vi "CSE ISP - options.vi"(8 "cmd":enum16{"get", "default"}(ring), 9 "enable menu (T)":bool=TRUE, 10 "item subtag":string, 11 "ISP menu":refnum<k9>) -> (0 "error out":errorcluster, 1 "VM params":T2, 2 "load FuncVIs":u32(ring)=2 items=["don't load", "load", "load & test"], 3 "dup ISP menu":refnum<k9>, 4 "Parse params":T4={"AutoParse"=TRUE, "GroupStm"=FALSE, "ErrSrcMaxLen"=180}, 5 "test syntax only":bool, 6 "misc params":T1, 7 "Exec params":T3={"pause counter"=1000, "pause, ms"=0, "autoVar"=TRUE, "enCpx"=TRUE})   [LabVIEW 2021]
doc: "::: CalcExpress Toolkit :::\nCopyright (c) 2000-2026 Konstantin Shifershteyn. All rights reserved."
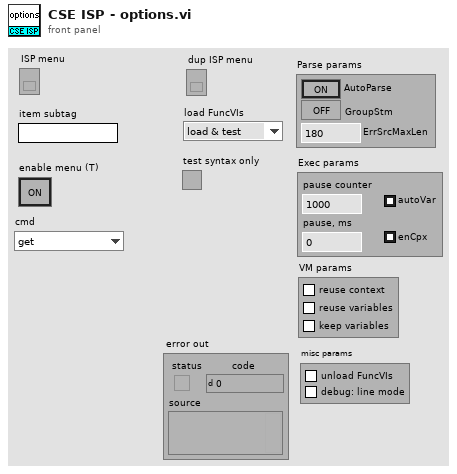
[diagram p1: front panel]
types:
  T1 = cluster{"unload FuncVIs":bool, "debug: line mode":bool}
  T2 = cluster{"reuse context":bool, "reuse variables":bool, "keep variables":bool}
  T3 = cluster{"pause counter":i32, "pause, ms":i32, "autoVar":bool, "enCpx":bool}
  T4 = cluster{"AutoParse":bool, "GroupStm":bool, "ErrSrcMaxLen":i32}
  T5 = cluster{i32, i32, "checked":bool, "checked":bool}
  T6 = cluster{"checked":bool, "checked":bool, "checked":bool}
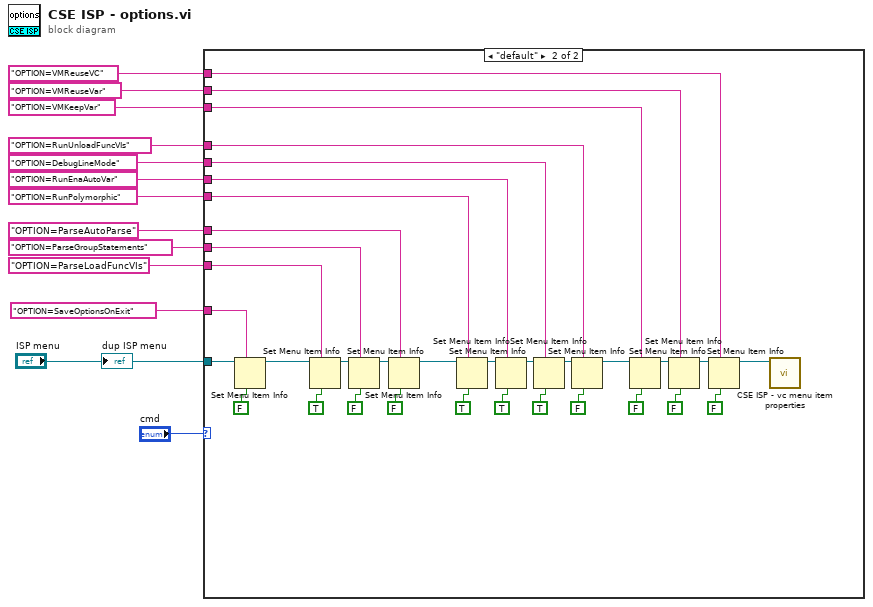
[diagram p0: block diagram]
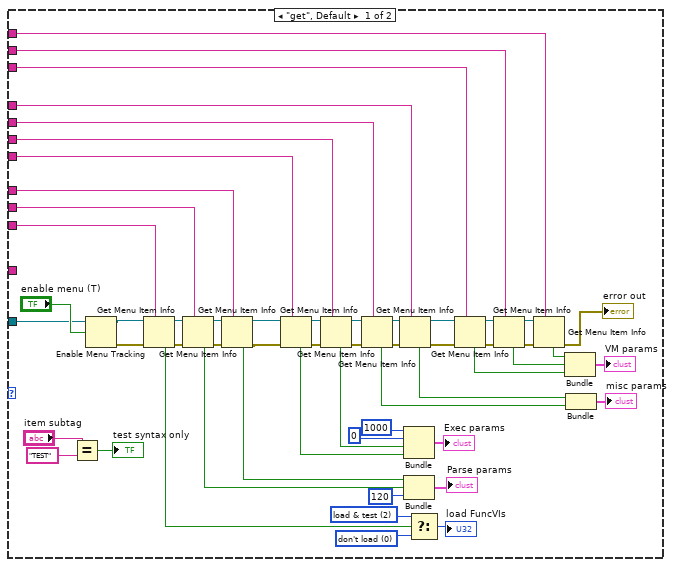
[diagram p2: hidden frame]
diagram:
  n1 = case shown="\"default\"" "cmd" {
    tunnel: "OPTION=RunUnloadFuncVIs" ("item tag") -> [w69 w103]
    tunnel: "OPTION=ParseGroupStatements" ("item tag") -> [w67 w101]
    tunnel: "OPTION=ParseAutoParse" ("item tag") -> [w66 w100]
    tunnel: "OPTION=RunPolymorphic" ("item tag") -> [w56 w99]
    tunnel: "OPTION=RunEnaAutoVar" ("item tag") -> [w55 w98]
    tunnel: "OPTION=ParseLoadFuncVIs" ("item tag") -> [w50 w102]
    tunnel: "ISP menu" -> [w43 w77]
    tunnel: "OPTION=SaveOptionsOnExit" ("item tag") -> [_ w87]
    tunnel: "OPTION=VMReuseVC" ("item tag") -> [w35 w81]
    tunnel: "OPTION=VMReuseVar" ("item tag") -> [w34 w82]
    tunnel: "OPTION=VMKeepVar" ("item tag") -> [w33 w83]
    tunnel: "OPTION=DebugLineMode" ("item tag") -> [w23 w73]
    frame "get", Default {
      w44 = u32 2 items=["don't load", "load", "load & test"] ("load FuncVIs")
      w45 = u32 0 items=["don't load", "load", "load & test"] ("load FuncVIs")
      n2 = Equal?(x="item subtag", y="TEST") -> (x = y?=→"test syntax only":bool)
      n3 = Enable Menu Tracking(3:"enable menu (T)", 4:w43) -> (0:w29:errorcluster, 1:w30:refnum<k9>)  [unwired: 1 in]
      n4 = Get Menu Item Info(7:w50, 8:w29, 11:w30) -> (0:w48:errorcluster, 3:w49:refnum<k9>, 4:w47:bool)  [unwired: 4 out]
      n5 = Get Menu Item Info(7:w67, 8:w48, 11:w49) -> (0:w58:errorcluster, 3:w68:refnum<k9>, 4:w63:bool)  [unwired: 4 out]
      n6 = Get Menu Item Info(7:w66, 8:w58, 11:w68) -> (0:w14:errorcluster, 3:w15:refnum<k9>, 4:w64:bool)  [unwired: 4 out]
      n7 = Get Menu Item Info(7:w56, 8:w14, 11:w15) -> (0:w57:errorcluster, 3:w59:refnum<k9>, 4:w52:bool)  [unwired: 4 out]
      n8 = Get Menu Item Info(7:w55, 8:w57, 11:w59) -> (0:w25:errorcluster, 3:w24:refnum<k9>, 4:w53:bool)  [unwired: 4 out]
      n9 = Get Menu Item Info(7:w23, 8:w25, 11:w24) -> (0:w18:errorcluster, 3:w19:refnum<k9>, 4:w21:bool)  [unwired: 4 out]
      n10 = Get Menu Item Info(7:w69, 8:w18, 11:w19) -> (0:w17:errorcluster, 3:w16:refnum<k9>, 4:w22:bool)  [unwired: 4 out]
      n11 = Bundle(1000, 0, "checked"=w53, "checked"=w52) -> (→"Exec params":T5)  [unwired: 1 in]
      n12 = Bundle("checked"=w64, "checked"=w63, 120) -> (→"Parse params":cluster{"checked":bool, "checked":bool, i32})  [unwired: 1 in]
      n13 = Select(t=w44, s=w47, f=w45) -> (s? t:f=→"load FuncVIs":u32)
      n14 = Get Menu Item Info(7:w33, 8:w17, 11:w16) -> (0:w40:errorcluster, 3:w42:refnum<k9>, 4:w36:bool)  [unwired: 4 out]
      n15 = Get Menu Item Info(7:w34, 8:w40, 11:w42) -> (0:w39:errorcluster, 3:w41:refnum<k9>, 4:w37:bool)  [unwired: 4 out]
      n16 = Get Menu Item Info(7:w35, 8:w39, 11:w41) -> (0:→"error out":errorcluster, 4:w38:bool)  [unwired: 5 out]
      n17 = Bundle("checked"=w38, "checked"=w37, "checked"=w36) -> (→"VM params":T6)  [unwired: 1 in]
      n18 = Bundle("checked"=w22, "checked"=w21) -> (→"misc params":cluster{"checked":bool, "checked":bool})  [unwired: 1 in]
    }
    frame "default" {
      n19 = Set Menu Item Info(6:FALSE ("checked"), 7:w87, 11:w77) -> (3:w76:refnum<k9>)  [unwired: 4 in, 1 out]
      n20 = Set Menu Item Info(6:TRUE ("checked"), 7:w102, 11:w76) -> (3:w97:refnum<k9>)  [unwired: 4 in, 1 out]
      n21 = Set Menu Item Info(6:FALSE ("checked"), 7:w101, 11:w97) -> (3:w96:refnum<k9>)  [unwired: 4 in, 1 out]
      n22 = Set Menu Item Info(6:FALSE ("checked"), 7:w100, 11:w96) -> (3:w71:refnum<k9>)  [unwired: 4 in, 1 out]
      n23 = Set Menu Item Info(6:TRUE ("checked"), 7:w99, 11:w71) -> (3:w95:refnum<k9>)  [unwired: 4 in, 1 out]
      n24 = Set Menu Item Info(6:TRUE ("checked"), 7:w98, 11:w95) -> (3:w74:refnum<k9>)  [unwired: 4 in, 1 out]
      n25 = Set Menu Item Info(6:TRUE ("checked"), 7:w73, 11:w74) -> (3:w72:refnum<k9>)  [unwired: 4 in, 1 out]
      n26 = Set Menu Item Info(6:FALSE ("checked"), 7:w103, 11:w72) -> (3:w70:refnum<k9>)  [unwired: 4 in, 1 out]
      n27 = Set Menu Item Info(6:FALSE ("checked"), 7:w83, 11:w70) -> (3:w79:refnum<k9>)  [unwired: 4 in, 1 out]
      n28 = Set Menu Item Info(6:FALSE ("checked"), 7:w82, 11:w79) -> (3:w80:refnum<k9>)  [unwired: 4 in, 1 out]
      n29 = Set Menu Item Info(6:FALSE ("checked"), 7:w81, 11:w80) -> (3:w78:refnum<k9>)  [unwired: 4 in, 1 out]
      n30 = call "CSE ISP - vc menu item properties.vi"("ISP menu"=w78) -> ()  [unwired: 7 in, 2 out]
    }
  }
  "dup ISP menu" <- "ISP menu"
